vi "ValueChangeTrigger.vi"(9 "新值":variant, 10 "控件引用":refnum<vi>) -> ()   [LabVIEW 2025]
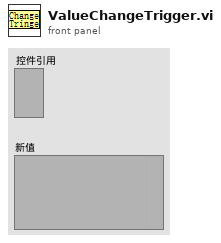
[diagram p1: front panel]
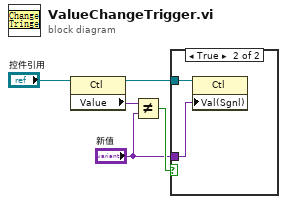
[diagram p0: block diagram]
diagram:
  n1 = property class="Ctl"(reference="控件引用") -> (reference out=w1:refnum<vi>, "Value"=w4:variant)  [unwired: 1 in, 1 out]
  n2 = Not Equal?(x=w4, y="新值") -> (x != y?=w3:bool)
  n3 = case shown="True" w3 {
    tunnel: "新值" -> [_ w6]
    tunnel: w1 -> [_ w7]
    frame False {
    }
    frame True {
      n4 = property class="Ctl"(reference=w7, "Val(Sgnl)"=w6) -> ()  [unwired: 1 in, 2 out]
    }
  }
